vi "Write XML Document.vi"(8 "error in (no error)":errorcluster, 10 "XML Document":refnum<k24>, 11 "ToastFromXML in":refnum<class "ToastFromXML.lvclass">) -> (0 "error out":errorcluster, 3 "ToastFromXML out":refnum<class "ToastFromXML.lvclass">)   [LabVIEW 2026, in "ToastNotification.lvlib" / "ToastFromXML.lvclass"]
doc: "Store the private XML Document reference through the class property. Skipped on incoming error. Does not clone or close the previous document. Internal ownership assignment used during construction; the source owner later calls Close."
uses:
  ToastFromXML.lvclass
  ToastFromXML.lvclass/ToastFromXML.ctl
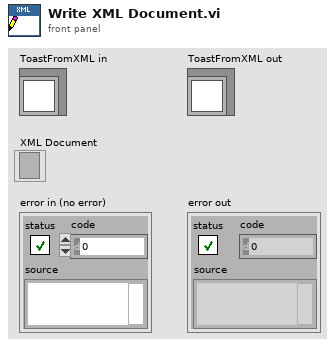
[diagram p1: front panel]
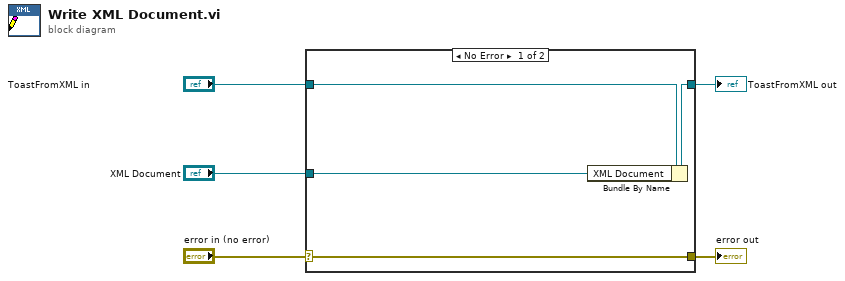
[diagram p0: block diagram]
diagram:
  n1 = case shown="No Error" "error in (no error)" {
    selector: "error in (no error)" -> [w9 w10]
    tunnel: [w9 w10] -> w4
    tunnel: [w7 w11] -> w2
    tunnel: "ToastFromXML in" -> [w8 w11]
    tunnel: "XML Document" -> [w6 _]
    frame No Error {
      n2 = Bundle By Name(cluster=w8, "XML Document"=w6) -> (w7:refnum<class "ToastFromXML.lvclass">)
    }
    frame Error {
    }
  }
  "error out" <- w4
  "ToastFromXML out" <- w2
